vi "upload_to_s3.vi"(8 "error in":errorcluster, 10 "File":path, 11 "Nominal Client in":refnum<class "Nominal Client.lvclass">) -> (0 "error out":errorcluster, 2 "source":refnum<class "s3.lvclass">, 3 "Nominal Client out":refnum<class "Nominal Client.lvclass">)   [LabVIEW 2020, in "Nominal Client.lvclass"]
doc: "Uploads a file to Nominal by taking the file path as input and automatically selecting the appropriate upload technique based on the file size. Small files are uploaded in a single operation, while large files are uploaded using a multipart strategy for efficiency and reliability."
uses:
  Nominal Client.lvclass
  datasources/s3/s3.lvclass
  datasources/source/create_s3.vi
  datasources/source/source.lvclass
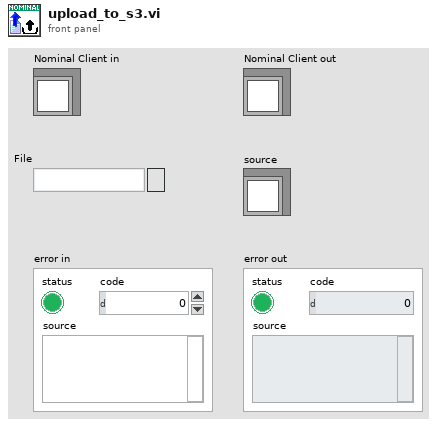
[diagram p1: front panel]
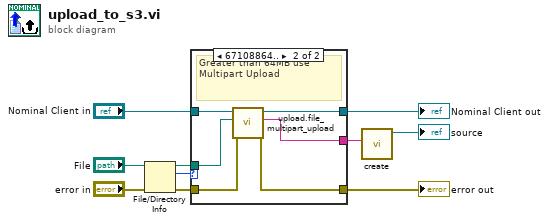
[diagram p0: block diagram]
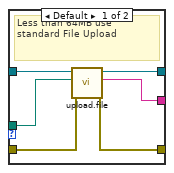
[diagram p2: hidden frame]
diagram:
  n1 = File/Directory Info(path="File", error in="error in") -> (path out=w7:path, size=w9:i64, error out=w4:errorcluster)  [unwired: 4 out]
  n2 = case shown="67108864.." w9 {
    tunnel: w7 -> [w16 w19]
    tunnel: "Nominal Client in" -> [w15 w22]
    tunnel: [w14 w21] -> w5
    tunnel: w4 -> [w13 w18]
    tunnel: [w12 w17] -> w3
    tunnel: [w11 w20] -> w2
    frame Default {
      # "Less than 64MB use standard File Upload"
      n3 = call "upload.file.vi"("error in"=w13, "File"=w16, "Nominal Client in"=w15) -> ("error out"=w12:errorcluster, "Path to S3 File"=w11:string, "Nominal Client out"=w14:refnum<class "Nominal Client.lvclass">)  [unwired: 6 in]
    }
    frame 67108864.. {
      # "Greater than 64MB use Multipart Upload"
      n4 = call "upload.file_multipart_upload.vi"("error in"=w18, "File Path"=w19, "Nominal Client in"=w22) -> ("error out"=w17:errorcluster, "S3 Path to File"=w20:string, "Nominal Client out"=w21:refnum<class "Nominal Client.lvclass">)  [unwired: 6 in]
    }
  }
  "Nominal Client out" <- w5
  "error out" <- w3
  n5 = call-poly "create.vi"("Path"=w2) -> ("source"=→"source":refnum<class "s3.lvclass">)  [unwired: 10 in]
